vi "Get Start Time.vi"(8 "error in (no error)":errorcluster, 11 "XNET CAN RW in":refnum<class "XNET CAN RW.lvclass">) -> (0 "error out":errorcluster, 3 "XNET CAN RW out":refnum<class "XNET CAN RW.lvclass">)   [LabVIEW 2021, in "XNET CAN RW.lvclass"]
uses:
  XNET CAN RW.lvclass
  XNET CAN RW.lvclass/XNET CAN RW.ctl
  typedef/Errors.ctl
  <vilib>/xnet/xnet.llb/XNET Read (State Time Start).vi
  Add Error Core.vi
  <vilib>/CIF Foundation/CIF Utilities/Time/Time_CIF_U.lvlib
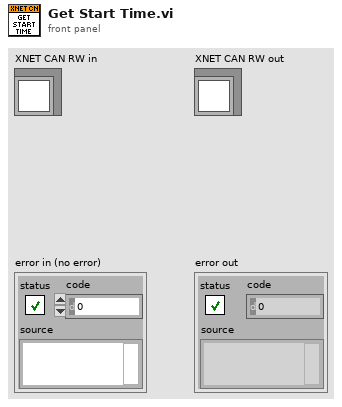
[diagram p1: front panel]
types:
  T1 = typedef "XNET CAN RW.lvclass/Errors.ctl" = enum16{"TX Timeout", "Packet Length", "Invalid Start Time"}
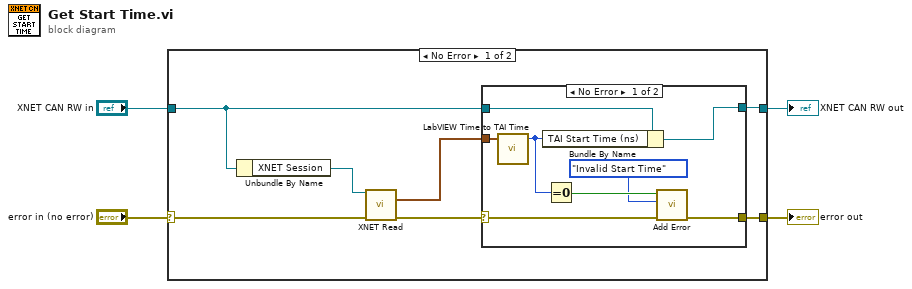
[diagram p0: block diagram]
diagram:
  n1 = case shown="No Error" "error in (no error)" {
    selector: "error in (no error)" -> [w9 w23]
    tunnel: [w5 w23] -> w3
    tunnel: [w7 w22] -> w1
    tunnel: "XNET CAN RW in" -> [w8 w22]
    frame No Error {
      n2 = Unbundle By Name(w8) -> ("XNET Session"=w11:refnum<k21>)
      n3 = call-poly <vilib>:"XNET Read.vi"("session in"=w11, "error in (no error)"=w9) -> ("local time start"=w10:timestamp, "error out"=w6:errorcluster)  [unwired: 9 in, 3 out]
      n4 = case shown="No Error" w6 {
        selector: w6 -> [w15 w20]
        tunnel: w10 -> [w19 _]
        tunnel: w8 -> [w18 w21]
        tunnel: [w17 w21] -> w7
        tunnel: [w14 w20] -> w5
        frame No Error {
          n5 = call <vilib>:"LabVIEW Time to TAI Time.vi"("LabVIEW Time (s)"=w19) -> ("TAI Time (ns)"=w16:i64)  [unwired: 4 in]
          n6 = Bundle By Name(cluster=w18, "TAI Start Time (ns)"=w16) -> (w17:refnum<class "XNET CAN RW.lvclass">)
          n7 = Equal To 0?(x=w16) -> (x = 0?=w13:bool)
          n8 = call "Add Error.vi"("error in (no error)"=w15, "Error"=Errors."Invalid Start Time", "Insert Error"=w13) -> ("error out"=w14:errorcluster)  [unwired: 8 in]
        }
        frame Error {
        }
      }
    }
    frame Error {
    }
  }
  "error out" <- w3
  "XNET CAN RW out" <- w1
